vi "Check_Interlock_status.vi"(8 "error in":errorcluster, 11 "VISA resource name":refnum<visa-resource-name>) -> (0 "error out":errorcluster, 3 "RESULT":bool)   [LabVIEW 2021]
uses:
  HI-POT_Driver/GPT-9800_GSB_L8.5/GPT-9000.lvlib
panel:
  out "Return  the test status":string
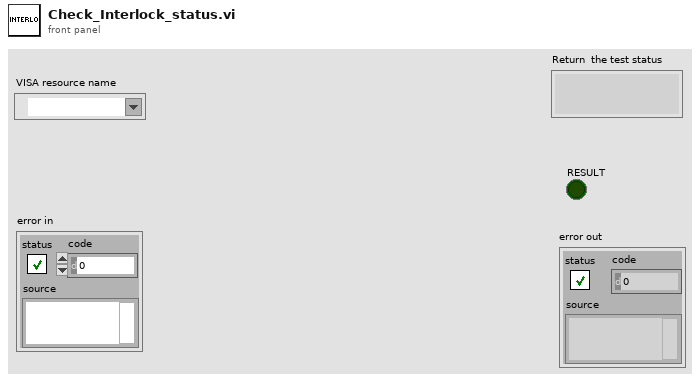
[diagram p1: front panel]
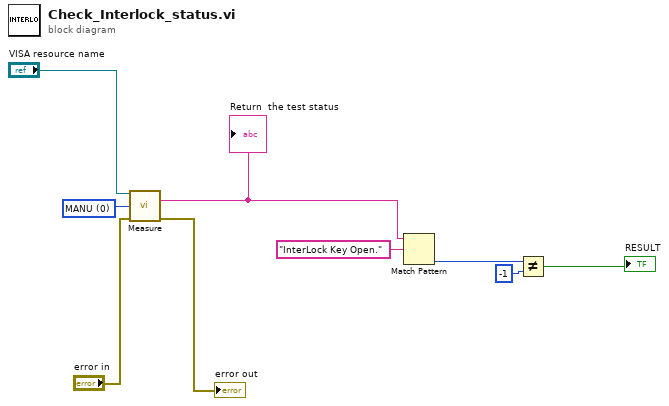
[diagram p0: block diagram]
diagram:
  w6 = u8 0 items=["MANU", "AUTO"] ("Function Mode Numeric")
  n1 = call "Measure.vi"("VISA resource name"="VISA resource name", "Function Mode Numeric"=w6, "error in"="error in") -> ("Return  the test status"=w1:string, "error out"=→"error out":errorcluster)  [unwired: 9 in, 2 out]
  "Return  the test status" <- w1
  n2 = Match Pattern(string=w1, regular expression="InterLock Key Open.") -> (offset past match=w8:i32)  [unwired: 1 in, 3 out]
  n3 = Not Equal?(x=w8, y=-1) -> (x != y?=→"RESULT":bool)
